vi "XPN Auto Load Calibration.vi"(8 "error in (no error)":errorcluster, 10 "gainLoaded":i32, 11 "offsetLoaded":i32) -> (0 "error out":errorcluster, 1 "function return":i32, 2 "gainLoaded out":i32, 3 "offsetLoaded out":i32)   [LabVIEW 2022 SP3, in "xPanelWrapper.lvlib"]
doc: "XPN_API int XPN_AutoLoadCalibration(int* offsetLoaded, int* gainLoaded);"
uses:
  xPanelWrapper.lvlib
  xPanelWrapper.dll
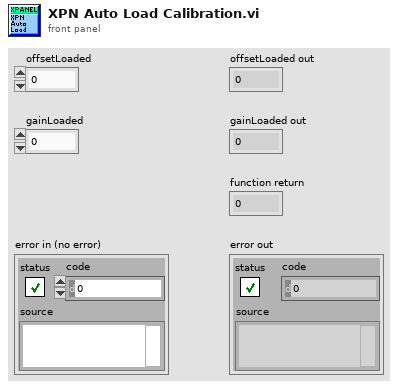
[diagram p1: front panel]
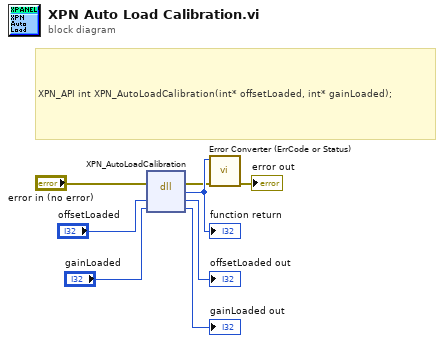
[diagram p0: block diagram]
diagram:
  # "XPN_API int XPN_AutoLoadCalibration(int* offsetLoaded, int* gainLoaded);"
  n1 = dll-call lib="E:/SourceCodes/image-harvest/ImageHandler/xPanelWrapperLvLib/xPanelWrapper.*" fn="XPN_AutoLoadCalibration"(error in="error in (no error)", "offsetLoaded"="offsetLoaded", "gainLoaded"="gainLoaded") -> (error out=w2:errorcluster, w8:i32, "offsetLoaded"=→"offsetLoaded out":i32, "gainLoaded"=→"gainLoaded out":i32)  [unwired: 2 in, 1 out]
  "function return" <- w8
  n2 = call "Error Converter (ErrCode or Status).vi"("error in (no error)"=w2, "error code"=w8) -> ("error out"=→"error out":errorcluster)  [unwired: 9 in]
